vi "Remove Project.vi"(7 "Project Store in":refnum<class "Project Store.lvclass">, 8 "error in (no error)":errorcluster, 11 "ID":string) -> (0 "error out":errorcluster, 3 "found?":bool, 5 "Project Store out":refnum<class "Project Store.lvclass">)   [LabVIEW 2024, in "Project Store.lvclass"]
doc: "Removes the project with the given ID and every task that belongs to it from the in-memory model. found? is FALSE when no project has that ID (its tasks are still removed if any exist). Nothing is written to disk until Write to Data Source.\n\nGenerated by: Claude"
uses:
  Project Store.lvclass
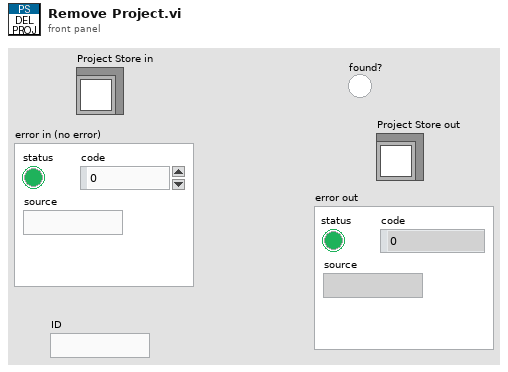
[diagram p1: front panel]
types:
  T1 = typedef "Project List.ctl" = T2[]
  T2 = typedef "Project.ctl" = cluster{"ID":string, "Name":string, "Active":bool, "Sort Order":i32}
  T3 = typedef "Task List.ctl" = T4[]
  T4 = typedef "Task.ctl" = cluster{"ID":string, "Project ID":string, "Name":string, "Active":bool, "Sort Order":i32}
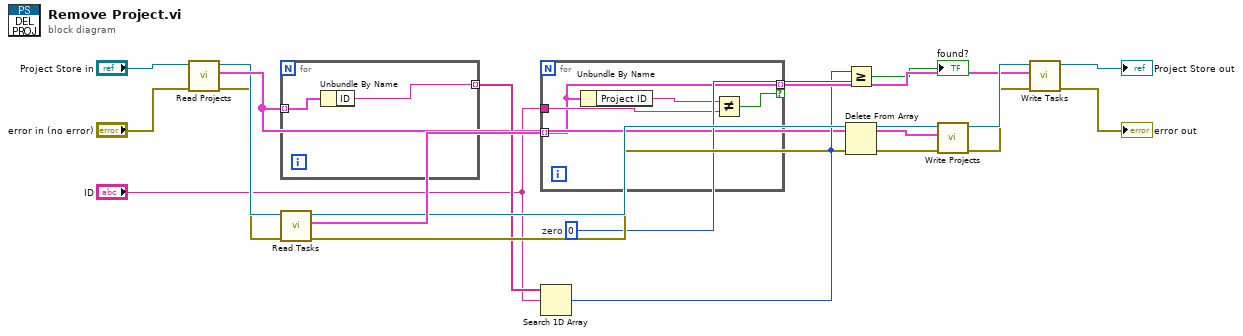
[diagram p0: block diagram]
diagram:
  w9 = 0  # zero
  n1 = call-dynamic "Read Projects.vi"("error in (no error)"="error in (no error)", "Project Store in"="Project Store in") -> ("error out"=w4:errorcluster, "Project List"=w6:T1, "Project Store out"=w5:refnum<class "Project Store.lvclass">)  [unwired: 7 in]
  n2 = for {
    tunnel: w6 -> [w20] mode=indexing
    tunnel: [w21] -> w7 mode=indexing
    n3 = Unbundle By Name(w20) -> ("ID"=w21:string)
  }
  n4 = call-dynamic "Read Tasks.vi"("error in (no error)"=w4, "Project Store in"=w5) -> ("error out"=w12:errorcluster, "Task List"=w14:T3, "Project Store out"=w13:refnum<class "Project Store.lvclass">)  [unwired: 7 in]
  n5 = for {
    tunnel: "ID" -> [w23]
    tunnel: w14 -> [w22] mode=indexing
    tunnel: [w22] -> w15 mode=indexing if=w25
    n6 = Unbundle By Name(w22) -> ("Project ID"=w24:string)
    n7 = Not Equal?(x=w24, y=w23) -> (x != y?=w25:bool)
  }
  n8 = Search 1D Array(1D array=w7, element="ID") -> (index of element=w8:i32)  [unwired: 1 in]
  n9 = Greater Or Equal?(x=w8, y=w9) -> (x >= y?=→"found?":bool)
  n10 = Delete From Array(array=w6, index=w8) -> (array with subset deleted=w11:T1)  [unwired: 1 in, 1 out]
  n11 = call-dynamic "Write Projects.vi"("error in (no error)"=w12, "Project List"=w11, "Project Store in"=w13) -> ("error out"=w16:errorcluster, "Project Store out"=w17:refnum<class "Project Store.lvclass">)  [unwired: 7 in]
  n12 = call-dynamic "Write Tasks.vi"("error in (no error)"=w16, "Task List"=w15, "Project Store in"=w17) -> ("error out"=→"error out":errorcluster, "Project Store out"=→"Project Store out":refnum<class "Project Store.lvclass">)  [unwired: 7 in]
